vi "Check Is Helper Already Running (Get Queue) -- Wrapper.vi"(7 "Create? (F: Check)":bool, 8 "error in (no error)":errorcluster, 11 "JKI SM in":refnum<class "JKI SM.lvclass">) -> (0 "error out":errorcluster, 2 "is Running?":bool)   [LabVIEW 2020]
uses:
  JKI State Machine API/source/JKI SM/JKI SM.lvclass
  JKI State Machine API/source/JKI SM/JKI SM.lvclass/JKI SM.ctl
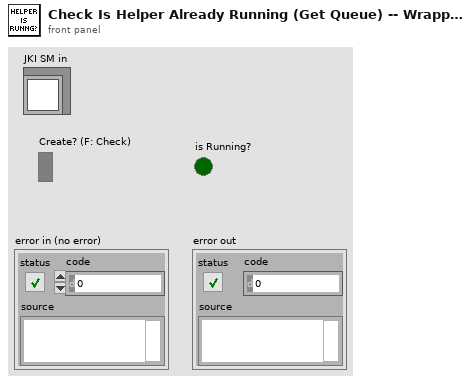
[diagram p1: front panel]
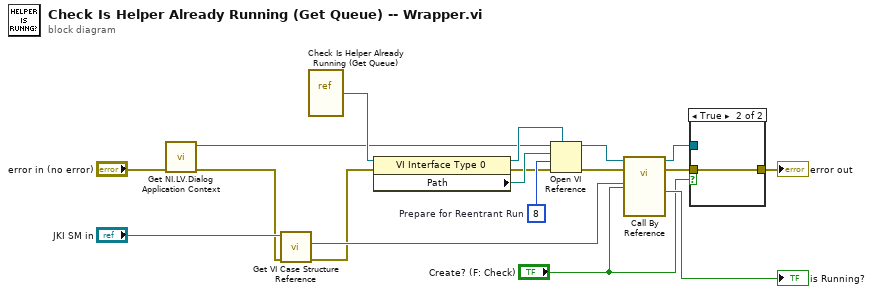
[diagram p0: block diagram]
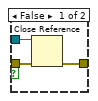
[diagram p2: hidden frame]
diagram:
  w17 = 8  # Prepare for Reentrant Run
  n1 = call "Get NI.LV.Dialog Application Context.vi"("error in (no error)"="error in (no error)") -> ("error out"=w3:errorcluster, "Application out"=w6:refnum<vi>)  [unwired: 9 in]
  n2 = call "Get VI Case Structure Reference.vi"("error in (no error)"=w3, "JKI SM in"="JKI SM in") -> ("error out"=w2:errorcluster, "Case Structure ref"=w5:refnum<vi>)  [unwired: 7 in, 1 out]
  n3 = vi-ref "Check Is Helper Already Running (Get Queue).vi"() -> (w18:refnum<vi>)
  n4 = property class="VI Interface Type 0"(reference=w18, error in=w2) -> (reference out=w13:refnum<vi>, error out=w8:errorcluster, "Path"=w16:path)
  n5 = Open VI Reference(type specifier VI Refnum (for type only)=w13, application reference (local)=w6, vi path=w16, options=w17, error in (no error)=w8) -> (vi reference=w15:refnum<vi>, error out=w14:errorcluster)  [unwired: 1 out]
  n6 = call-by-ref "?"(reference=w15, error in=w14, "Create? (F: Check)"="Create? (F: Check)", "GObject in"=w5) -> (reference out=w11:refnum<vi>, error out=w12:errorcluster, "is Running?"=→"is Running?":bool)  [unwired: 9 in]
  n7 = case shown="True" "Create? (F: Check)" {
    tunnel: w12 -> [w21 w22]
    tunnel: w11 -> [w20 _]
    tunnel: [w19 w22] -> w9
    frame False {
      n8 = Close Reference(reference=w20, error in (no error)=w21) -> (error out=w19:errorcluster)
    }
    frame True {
    }
  }
  "error out" <- w9
